vi "Speed_Command.vi"(8 "error in (no error)":errorcluster, 10 "Motor Control":dbl, 11 "Motor in":refnum<class "Motor.lvclass">) -> (0 "error out":errorcluster, 3 "Motor out":refnum<class "Motor.lvclass">)   [LabVIEW 2021, in "Motor.lvclass"]
uses:
  Motor.lvclass
  Motor.lvclass/Motor.ctl
  AnalogOutput/AnalogOutput.lvclass
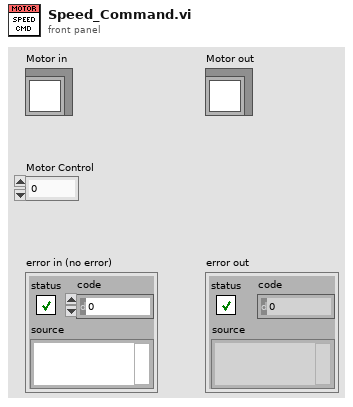
[diagram p1: front panel]
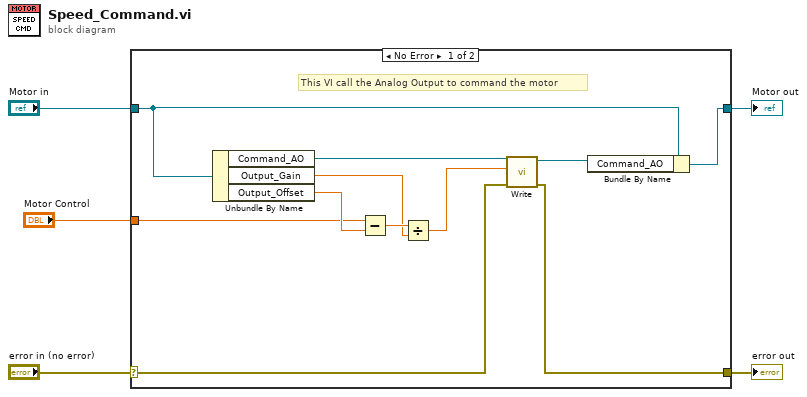
[diagram p0: block diagram]
diagram:
  n1 = case shown="No Error" "error in (no error)" {
    selector: "error in (no error)" -> [w15 w18]
    tunnel: [w14 w18] -> w4
    tunnel: [w11 w17] -> w2
    tunnel: "Motor in" -> [w12 w17]
    tunnel: "Motor Control" -> [w9 _]
    frame No Error {
      # "This VI call the Analog Output to command the motor"
      n2 = Unbundle By Name(w12) -> ("Command_AO"=w16:refnum<class "AnalogOutput.lvclass">, "Output_Gain"=w7:dbl, "Output_Offset"=w10:dbl)
      n3 = Subtract(x=w9, y=w10) -> (x-y=w8:dbl)
      n4 = Divide(x=w8, y=w7) -> (x/y=w6:dbl)
      n5 = call-dynamic "Write.vi"("error in (no error)"=w15, "data in"=w6, "AnalogOutput in"=w16) -> ("error out"=w14:errorcluster, "AnalogOutput out"=w13:refnum<class "AnalogOutput.lvclass">)  [unwired: 7 in]
      n6 = Bundle By Name(cluster=w12, "Command_AO"=w13) -> (w11:refnum<class "Motor.lvclass">)
    }
    frame Error {
    }
  }
  "error out" <- w4
  "Motor out" <- w2
